vi "scource and measeure.vi"() -> ()   [LabVIEW 2023]
panel:
  out "Y vs. Frequency":cluster{dbl, dbl}[](graph)
  in  "set reference value\n(no:f)":bool
  in  "measurement mode\n(LIN:f)":bool
  in  "detector selection\n(no change)":u16(ring) items=["no change", "rms", "average", "quasi-peak"]
  out "error out":errorcluster
  in  "measurements\n(AC level)":u16(ring) items=["AC level", "DC level", "Distortion", "Distortion level", "Signal-to-Noise", "SINAD"]
  out "value read 2":dbl format="%.7f"
  in  "stop":bool
  out "Waveform Chart":dbl[](graph)
  in  "error in (no error)":errorcluster
  in  "output impedence\n(f:60 ohms)":bool
  in  "source frequency\n(1000Hz)":dbl=1000.0 min=10.0 max=100000.0 format="%.5f"
  in  "frequency increment\n(1000Hz)":dbl=1000.0 format="%.5f"
  in  "amplitude increment\n(.1V)":dbl=0.1 format="%.5f"
  in  "source amplitude\n(.6mV)":dbl=0.0006 min=0.0006 max=6.0 format="%.5f"
  in  "SPCL 3 (special function 3)\npost-notch gain\n(auto select)":u16(ring) items=["automatic selection", "0dB", "20dB", "40dB", "60dB"]
  in  "SPCL 6(special funtion 6)\nnotch tune\n(false:automatic)":bool
  in  "SPCL 5(special funtion 5)\npost-notch detector response\n(fast rms) Except SINAD":u16(ring) items=["no change", "fast rms", "slow rms", "fast avg", "slow avg"]
  in  "HighPass/BandPass filter\n(off)":u16(ring) items=["off ", "left HP/BP filter", "right HP/BP filter"]
  in  "low pass filters\n(30kHz)":u16(ring)=1 items=["off(750kHz) ", "low pass 30kHz", "low pass 80 kHz"]
  in  "SINAD meter range\n(f:0 to 18)":bool
  in  "range selector\n(f:except DC)":bool
  in  "start frequency (Hz)":dbl=50.0 min=5.0 max=100000.0 format="%.5f"
  in  "stop frequency (Hz)":dbl=30000.0 min=20.0 max=100000.0 format="%.5f"
  in  "SPCL 17(special funtion 17)\nsweep resolution\n(5points/decade)":u16(ring)=2 items=["1 point/decade", "2 points/decade", "5 points/decade", "10 points/decade", "20 points/decade", "50 points/decade", "100 points/decade", "200 points/decade", "500 points/decade"]
  in  "SPCL 2(spcial function 2)\ninput level range(DC only)\n(auto select)":u16(ring) items=["automatic select", "300V", "64V", "16V", "4V"]
  in  "SPCL 2(spcial function 1)\ninput level range(except DC)\n(auto select)":u16(ring) items=["automatic select", "300V", "189V", "119V", "75.4V", "47.6V", "30.0V", "18.9V", "11.9V", "7.54V", "4.76V", "3.00V", "1.89V", "1.19V", "0.754V", "0.476V", "0.300V", "0.189V", "0.119V", "0.0754V"]
  in  "VISA resource name":refnum<visa-resource-name>
  # "0 to 24 dB"
  # "0 to 18 dB"
  # "input range (DC only)"
  # "input range (except DC)"
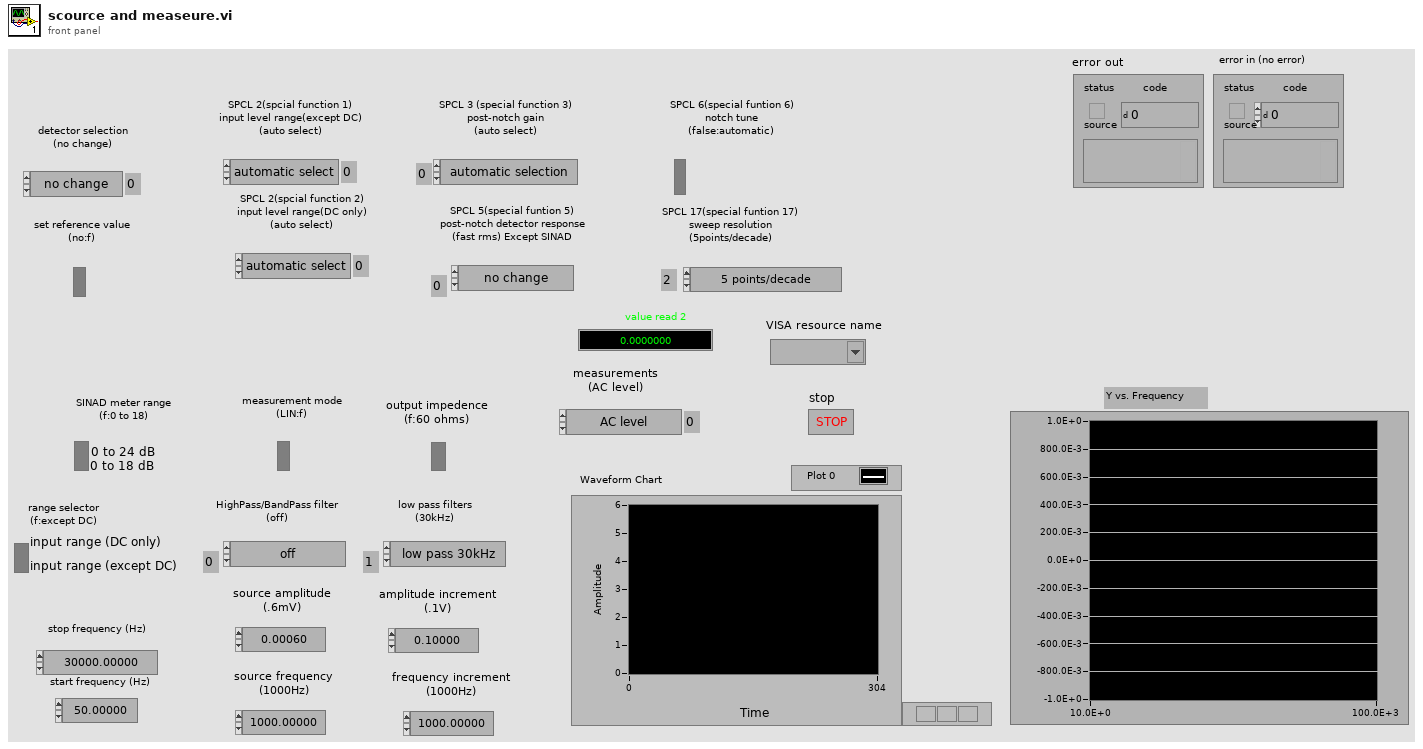
[diagram p1: front panel]
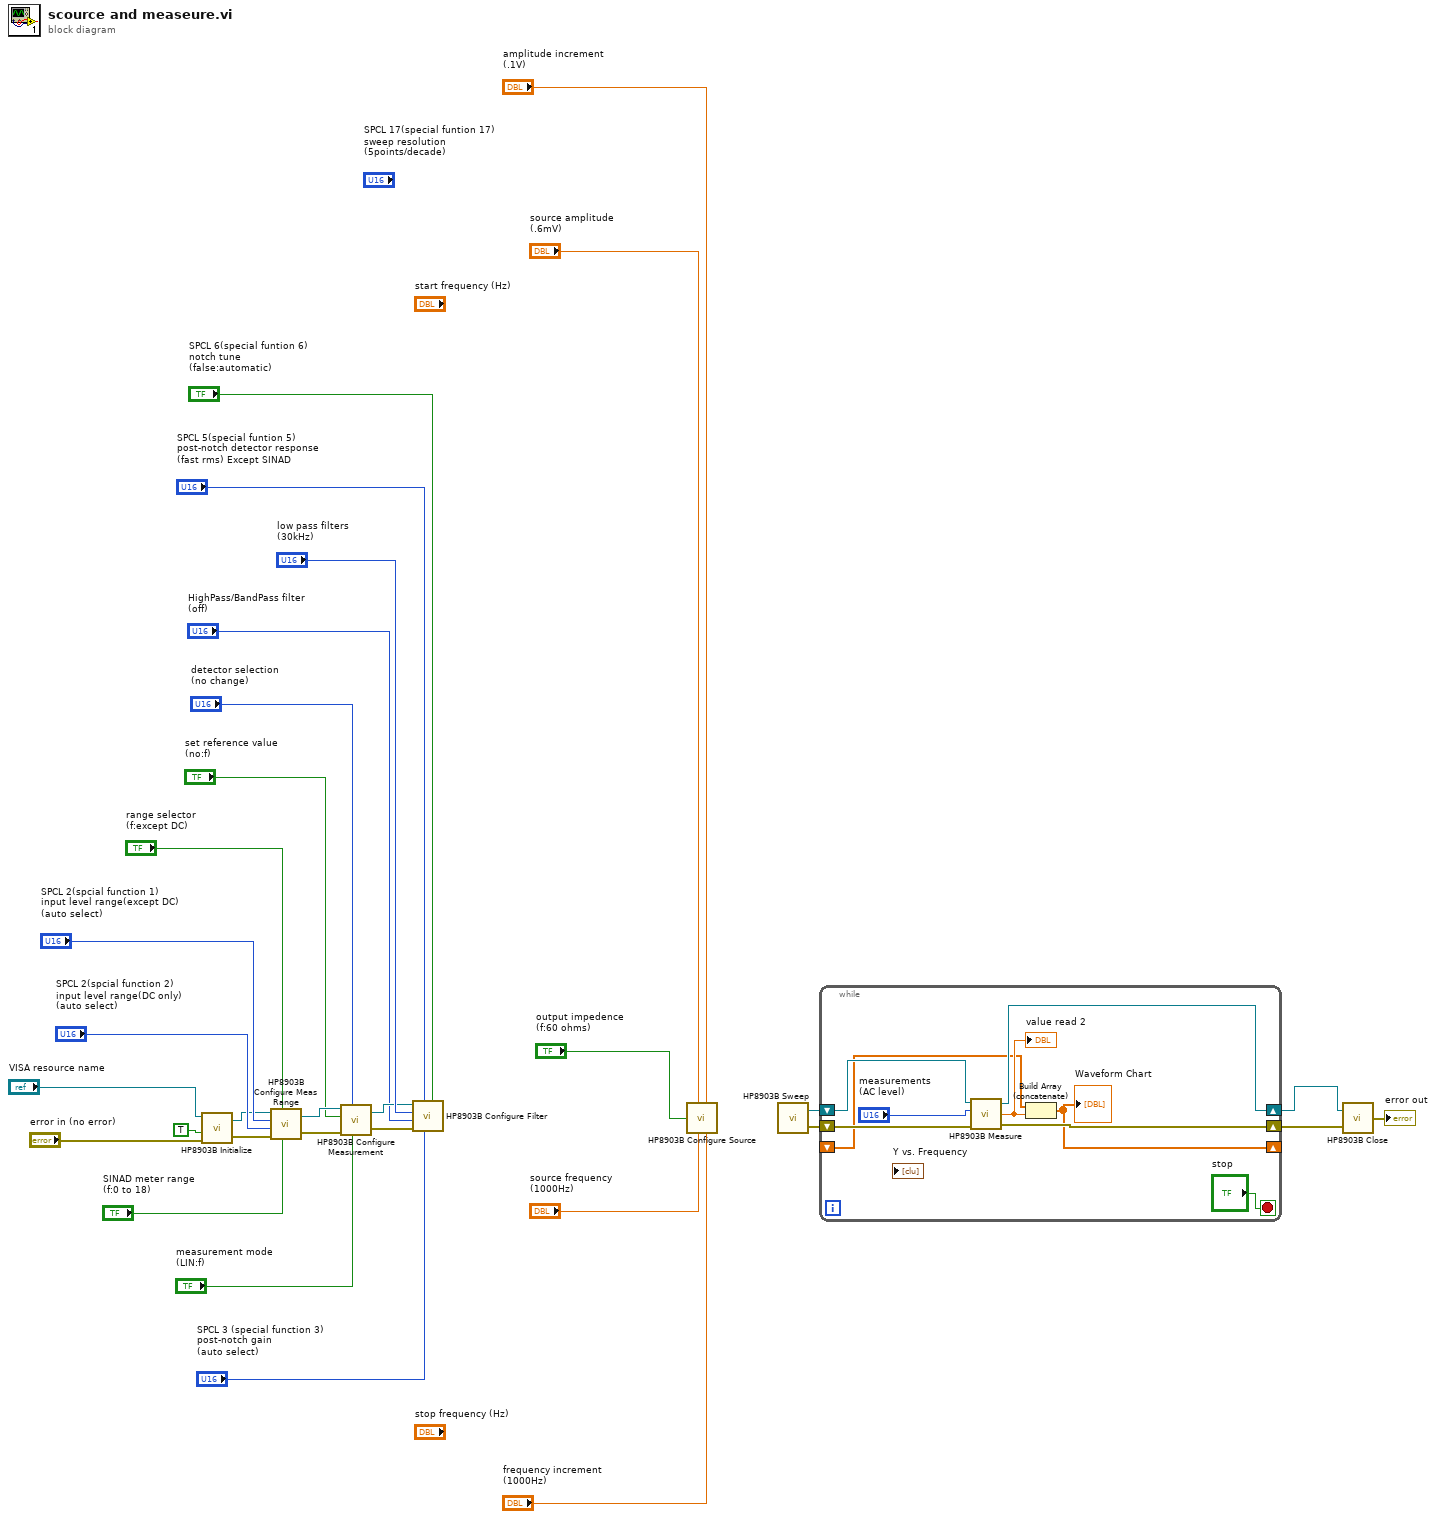
[diagram p0: block diagram]
diagram:
  n1 = call <instrlib>:"HP8903B Initialize.vi"("error in (no error)"="error in (no error)", "reset (no : F)"=TRUE, "VISA resource name"="VISA resource name") -> ("error out"=w28:errorcluster, "VISA session"=w29:refnum<visa-resource-name>)  [unwired: 1 in]
  n2 = call <instrlib>:"HP8903B Configure Meas Range.vi"("SINAD meter range\n(f:0 to 18)"="SINAD meter range\n(f:0 to 18)", "range selector\n(f:except DC)"="range selector\n(f:except DC)", "error in (no error)"=w28, "input level range : DC only\n(auto select)"="SPCL 2(spcial function 2)\ninput level range(DC only)\n(auto select)", "input level range : except DC\n(auto select)"="SPCL 2(spcial function 1)\ninput level range(except DC)\n(auto select)", "VISA session"=w29) -> ("error out"=w4:errorcluster, "dup VISA session"=w5:refnum<visa-resource-name>)
  n3 = call <instrlib>:"HP8903B Configure Measurement.vi"("measurement mode\n(LIN:f)"="measurement mode\n(LIN:f)", "detector selection\n(no change)"="detector selection\n(no change)", "error in (no error)"=w4, "set reference value\n(no:f)"="set reference value\n(no:f)", "VISA session"=w5) -> ("error out"=w9:errorcluster, "dup VISA session"=w8:refnum<visa-resource-name>)  [unwired: 1 in]
  n4 = call <instrlib>:"HP8903B Configure Filter.vi"("notch tune\n(false:automatic)"="SPCL 6(special funtion 6)\nnotch tune\n(false:automatic)", "post-notch gain\n(auto select)"="SPCL 3 (special function 3)\npost-notch gain\n(auto select)", "post-notch detector response\n(fast rms)"="SPCL 5(special funtion 5)\npost-notch detector response\n(fast rms) Except SINAD", "error in (no error)"=w9, "HP/BP filter\n(off)"="HighPass/BandPass filter\n(off)", "low pass filters\n(30kHz)"="low pass filters\n(30kHz)", "VISA session"=w8) -> ()  [unwired: 2 in, 2 out]
  n5 = call <instrlib>:"HP8903B Configure Source.vi"("source amplitude\n(.6mV)"="source amplitude\n(.6mV)", "output impedence\n(f:60 ohms)"="output impedence\n(f:60 ohms)", "source frequency\n(1000Hz)"="source frequency\n(1000Hz)", "amplitude increment\n(.1V)"="amplitude increment\n(.1V)", "frequency increment\n(1000Hz)"="frequency increment\n(1000Hz)") -> ()  [unwired: 4 in, 2 out]
  n6 = call <instrlib>:"HP8903B Sweep.vi"() -> ("error out"=w14:errorcluster, "dup VISA session"=w13:refnum<visa-resource-name>)  [unwired: 6 in]
  n7 = while {
    shift-right: [w39] -> w10
    shift-left: w14 -> [w43]
    shift-right: [w40] -> w11
    shift-left: w13 -> [w42]
    shift-right: [w35] -> _
    shift-left: _ -> [w36]
    stop <- "stop" stop-if-true
    n8 = call <instrlib>:"HP8903B Measure.vi"("error in (no error)"=w43, "measurements\n(AC level)"="measurements\n(AC level)", "VISA session"=w42) -> ("error out"=w39:errorcluster, "value read"=w37:dbl, "dup VISA session"=w40:refnum<visa-resource-name>)  [unwired: 1 in]
    "value read 2" <- w37
    n9 = Build Array (concatenate)(w36, w37) -> (w35:dbl[])
    "Waveform Chart" <- w35
  }
  n10 = call <instrlib>:"HP8903B Close.vi"("error in (no error)"=w10, "VISA session"=w11) -> ("error out"=→"error out":errorcluster)
